vi "Native_CreateControlVI.vi"() -> ()   [LabVIEW 2024]
panel:
  out "error out":errorcluster caption="错误输出"
  in  "output_path":path
  in  "vi_type":T1(ring)
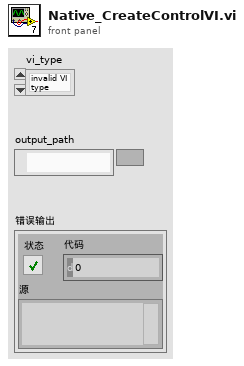
[diagram p1: front panel]
types:
  T1 = enum32{"invalid VI type", "Standard VI", "Control VI", "Global VI", "Polymorphic VI", "Configuration VI", "SubSystem", "Facade VI", "Method VI", "Statechart Diagram VI"}
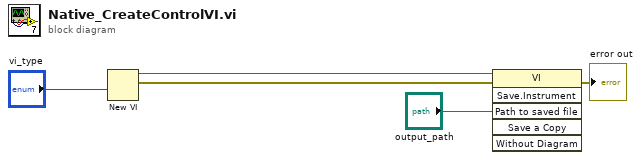
[diagram p0: block diagram]
diagram:
  n1 = New VI ("新建VI")(9:"vi_type") -> (0:w3:errorcluster, 3:w4:refnum<vi>)  [unwired: 6 in]
  n2 = invoke class="VI" method="Save.Instrument"(reference=w4, error in=w3, "Path to saved file"="output_path") -> (error out=→"error out":errorcluster)  [unwired: 3 in, 5 out]
